vi "Test_CLFN_Path_Cost.vi"() -> ()   [LabVIEW 2021]
uses:
  codec_vis/CANsub_Codec.lvlib
  libcansub_codec.dll
panel:
  out "median B - median A":dbl
  out "min A":dbl
  out "median A":dbl
  out "median B":dbl
  out "min B":dbl
  out "ret B":i32
  out "ret A":i32
  out "out_cap":i32
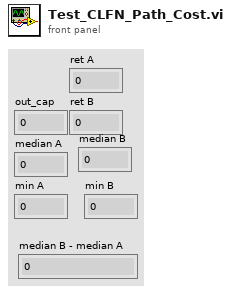
[diagram p1: front panel]
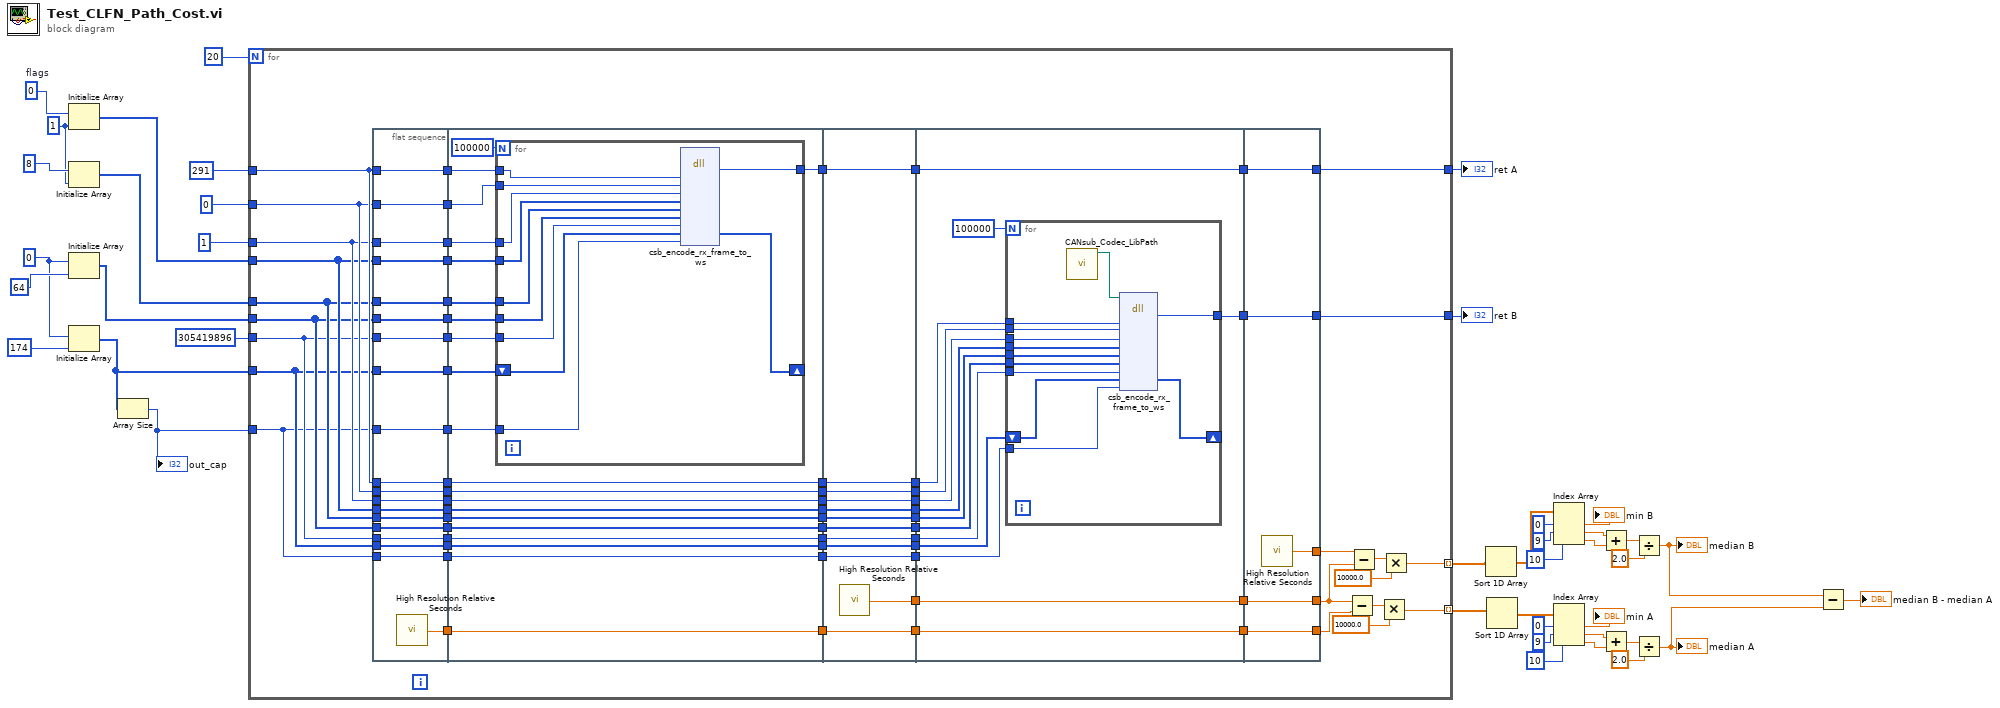
[diagram p0: block diagram]
diagram:
  w1 = u8 0
  w38 = 1 ("dimension size")
  w40 = u16 0  # flags
  n1 = Initialize Array(w40, w38) -> (w31:u16[])
  n2 = Initialize Array(u8 8, w38) -> (w30:u8[])
  n3 = Initialize Array(w1, 64 ("dimension size")) -> (w29:u8[])
  n4 = Initialize Array(w1, 174 ("dimension size")) -> (w28:u8[])
  n5 = Array Size(array=w28) -> (size(s)=w27:i32)
  "out_cap" <- w27
  n6 = for {
    N: 20 ("Iterations") -> [_]
    tunnel: u32 305419896 -> [w71]
    tunnel: u32 291 -> [w95]
    tunnel: 0 -> [w91]
    tunnel: 1 -> [w87]
    tunnel: w31 -> [w83]
    tunnel: w30 -> [w79]
    tunnel: w29 -> [w75]
    tunnel: w28 -> [w67]
    tunnel: w27 -> [w63]
    tunnel: [w49] -> w24 mode=indexing
    tunnel: [w48] -> w23 mode=indexing
    tunnel: [w47] -> w25
    tunnel: [w45] -> w26
    n7 = flat-sequence {
      tunnel: [w126] -> w107
      tunnel: w71 -> [w126]
      tunnel: [w125] -> w106
      tunnel: w95 -> [w125]
      tunnel: [w124] -> w105
      tunnel: w91 -> [w124]
      tunnel: [w123] -> w104
      tunnel: w87 -> [w123]
      tunnel: [w122] -> w103
      tunnel: w83 -> [w122]
      tunnel: w79 -> [w121]
      tunnel: [w121] -> w102
      tunnel: [w120] -> w101
      tunnel: w75 -> [w120]
      tunnel: [w119] -> w100
      tunnel: w67 -> [w119]
      tunnel: [w118] -> w99
      tunnel: w63 -> [w118]
      tunnel: [w117] -> w96
      tunnel: w95 -> [w117]
      tunnel: [w116] -> w92
      tunnel: w91 -> [w116]
      tunnel: [w115] -> w88
      tunnel: w87 -> [w115]
      tunnel: [w114] -> w84
      tunnel: w83 -> [w114]
      tunnel: [w113] -> w80
      tunnel: w79 -> [w113]
      tunnel: [w112] -> w76
      tunnel: w75 -> [w112]
      tunnel: [w111] -> w72
      tunnel: w71 -> [w111]
      tunnel: [w110] -> w68
      tunnel: w67 -> [w110]
      tunnel: [w109] -> w64
      tunnel: w63 -> [w109]
      tunnel: [w108] -> w57
      tunnel: w107 -> [w146]
      tunnel: w106 -> [w145]
      tunnel: w105 -> [w144]
      tunnel: w104 -> [w143]
      tunnel: w103 -> [w142]
      tunnel: w102 -> [w141]
      tunnel: w101 -> [w140]
      tunnel: w100 -> [w139]
      tunnel: w99 -> [w138]
      tunnel: [w137] -> w97
      tunnel: w96 -> [w137]
      tunnel: [w136] -> w93
      tunnel: w92 -> [w136]
      tunnel: [w135] -> w89
      tunnel: w88 -> [w135]
      tunnel: [w134] -> w85
      tunnel: w84 -> [w134]
      tunnel: [w133] -> w81
      tunnel: w80 -> [w133]
      tunnel: [w132] -> w77
      tunnel: w76 -> [w132]
      tunnel: [w131] -> w73
      tunnel: w72 -> [w131]
      tunnel: [w130] -> w69
      tunnel: w68 -> [w130]
      tunnel: [w129] -> w65
      tunnel: w64 -> [w129]
      tunnel: [w128] -> w58
      tunnel: w57 -> [w128]
      tunnel: [w127] -> w42
      tunnel: [w170] -> w98
      tunnel: w97 -> [w170]
      tunnel: [w169] -> w94
      tunnel: w93 -> [w169]
      tunnel: [w168] -> w90
      tunnel: w89 -> [w168]
      tunnel: [w167] -> w86
      tunnel: w85 -> [w167]
      tunnel: [w166] -> w82
      tunnel: w81 -> [w166]
      tunnel: [w165] -> w78
      tunnel: w77 -> [w165]
      tunnel: [w164] -> w74
      tunnel: w73 -> [w164]
      tunnel: [w163] -> w70
      tunnel: w69 -> [w163]
      tunnel: [w162] -> w66
      tunnel: w65 -> [w162]
      tunnel: [w161] -> w61
      tunnel: [w160] -> w59
      tunnel: w58 -> [w160]
      tunnel: [w159] -> w43
      tunnel: w42 -> [w159]
      tunnel: w98 -> [w183]
      tunnel: w94 -> [w182]
      tunnel: w90 -> [w181]
      tunnel: w86 -> [w180]
      tunnel: w82 -> [w179]
      tunnel: w78 -> [w178]
      tunnel: w74 -> [w177]
      tunnel: w70 -> [w176]
      tunnel: w66 -> [w175]
      tunnel: [w174] -> w62
      tunnel: w61 -> [w174]
      tunnel: [w173] -> w60
      tunnel: w59 -> [w173]
      tunnel: [w172] -> w46
      tunnel: [w171] -> w44
      tunnel: w43 -> [w171]
      tunnel: [w201] -> w50
      tunnel: w62 -> [w201]
      tunnel: [w200] -> w56
      tunnel: w60 -> [w200]
      tunnel: [w199] -> w51
      tunnel: [w198] -> w47
      tunnel: w46 -> [w198]
      tunnel: [w197] -> w45
      tunnel: w44 -> [w197]
      frame #0 {
        n8 = call <vilib>:"High Resolution Relative Seconds.vi"() -> ("relative seconds"=w108:dbl)
      }
      frame #1 {
        n9 = for {
          N: 100000 -> [_]
          tunnel: [w158] -> w127
          tunnel: w146 -> [w157]
          tunnel: w145 -> [w156]
          tunnel: w144 -> [w155]
          tunnel: w143 -> [w154]
          tunnel: w142 -> [w153]
          tunnel: w141 -> [w152]
          tunnel: w140 -> [w151]
          tunnel: w138 -> [w149]
          shift-right: [w148] -> _
          shift-left: w139 -> [w150]
          n10 = dll-call lib="libcansub_codec.*" fn="csb_encode_rx_frame_to_ws"("new_id"=w156, "index"=w155, "n_frames"=w154, "flags"=w153, "data_len"=w152, "data"=w151, "mask"=w157, "out"=w150, "out_cap"=w149) -> ("return type"=w158:i32, "out"=w148:u8[])  [unwired: 11 in, 2 out]
        }
      }
      frame #2 {
        n11 = call <vilib>:"High Resolution Relative Seconds.vi"() -> ("relative seconds"=w161:dbl)
      }
      frame #3 {
        n12 = for {
          N: 100000 -> [_]
          shift-right: [w195] -> _
          shift-left: w176 -> [w186]
          tunnel: [w194] -> w172
          tunnel: w183 -> [w193]
          tunnel: w182 -> [w192]
          tunnel: w181 -> [w191]
          tunnel: w180 -> [w190]
          tunnel: w179 -> [w189]
          tunnel: w178 -> [w188]
          tunnel: w177 -> [w187]
          tunnel: w175 -> [w185]
          n13 = call "CANsub_Codec_LibPath.vi"() -> ("Path"=w196:path)  [unwired: 11 in]
          n14 = dll-call lib="libcansub_codec.*" fn="csb_encode_rx_frame_to_ws"(path in=w196, "new_id"=w193, "index"=w192, "n_frames"=w191, "flags"=w190, "data_len"=w189, "data"=w188, "mask"=w187, "out"=w186, "out_cap"=w185) -> ("return type"=w194:i32, "out"=w195:u8[])  [unwired: 10 in, 2 out]
        }
      }
      frame #4 {
        n15 = call <vilib>:"High Resolution Relative Seconds.vi"() -> ("relative seconds"=w199:dbl)
      }
    }
    n16 = Subtract(x=w50, y=w56) -> (x-y=w55:dbl)
    n17 = Subtract(x=w51, y=w50) -> (x-y=w52:dbl)
    n18 = Multiply(x=w55, y=10000.0) -> (x*y=w48:dbl)
    n19 = Multiply(x=w52, y=10000.0) -> (x*y=w49:dbl)
  }
  "ret A" <- w26
  "ret B" <- w25
  n20 = Sort 1D Array(array=w24) -> (sorted array=w22:dbl[])
  n21 = Sort 1D Array(array=w23) -> (sorted array=w5:dbl[])
  n22 = Index Array(array=w22, index #1=0 ("index"), index #2=9 ("index"), index #3=10 ("index")) -> (element #1=→"min B":dbl, element #2=w17:dbl, element #3=w16:dbl)
  n23 = Index Array(array=w5, index #1=0 ("index"), index #2=9 ("index"), index #3=10 ("index")) -> (element #1=→"min A":dbl, element #2=w10:dbl, element #3=w11:dbl)
  n24 = Add(x=w17, y=w16) -> (x+y=w15:dbl)
  n25 = Add(x=w10, y=w11) -> (x+y=w12:dbl)
  n26 = Divide(x=w15, y=2.0) -> (x/y=w4:dbl)
  "median B" <- w4
  n27 = Divide(x=w12, y=2.0) -> (x/y=w3:dbl)
  "median A" <- w3
  n28 = Subtract(x=w4, y=w3) -> (x-y=→"median B - median A":dbl)
